vi "Echo_Handle_Frames_API.vi"(5 "frames":T1 {"flags" format="%.0x"; "id" format="%.0x"}, 7 "context":T2 {"ack hi" format="%.0x"; "ack lo" format="%.0x"; "test hi" format="%.0x"; "test lo" format="%.0x"}, 8 "error in (no error)":errorcluster, 9 "counters in":T3, 10 "time store in":T4, 11 "channel in":refnum<class "CANsub_Channel.lvclass">) -> (0 "error out":errorcluster, 1 "counters out":T3, 2 "time store out":T4, 3 "channel out":refnum<class "CANsub_Channel.lvclass">)   [LabVIEW 2021]
doc: "S5 echo via API: handles all frames of one Read: frames received += count; per frame Echo_Classify_API ? Test: Echo_Send_Echo_API, Ack: Echo_Send_Report, Other: nothing. Loop-safe: no allocation, bounded time."
uses:
  Echo_Time_Store.ctl
  Echo_Counters.ctl
  Echo_Context.ctl
  api/CANsub_Channel/CANsub_Channel.lvclass
  api/Typedefs/CANsub_Frames.ctl
  api/CANsub_API.lvlib
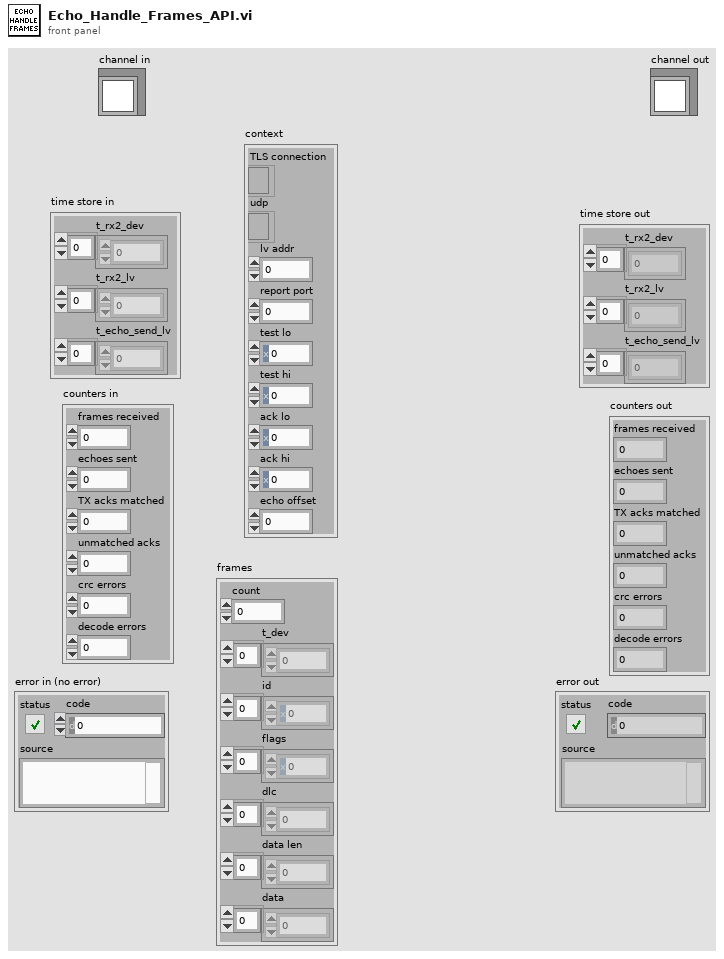
[diagram p1: front panel]
types:
  T1 = typedef "CANsub_API.lvlib/CANsub_Frames.ctl" = cluster{"count":i32, "t_dev":dbl[], "id":u32[], "flags":u16[], "dlc":u8[], "data len":u8[], "data":u8[]}
  T2 = typedef "Echo_Context.ctl" = cluster{"TLS connection":refnum<k5>, "udp":refnum<k16>, "lv addr":u32, "report port":u16, "test lo":u32, "test hi":u32, "ack lo":u32, "ack hi":u32, "echo offset":i32}
  T3 = typedef "Echo_Counters.ctl" = cluster{"frames received":u32, "echoes sent":u32, "TX acks matched":u32, "unmatched acks":u32, "crc errors":u32, "decode errors":i32}
  T4 = typedef "Echo_Time_Store.ctl" = cluster{"t_rx2_dev":dbl[], "t_rx2_lv":dbl[], "t_echo_send_lv":dbl[]}
  T5 = typedef "Echo_Frame.ctl" = cluster{"kind":T6, "id":u32, "t_dev":dbl, "seq":u16, "idx":u8, "key":i32, "index":i32}
  T6 = typedef "Echo_Frame_Kind.ctl" = enum16{"Other", "Test", "Ack"}
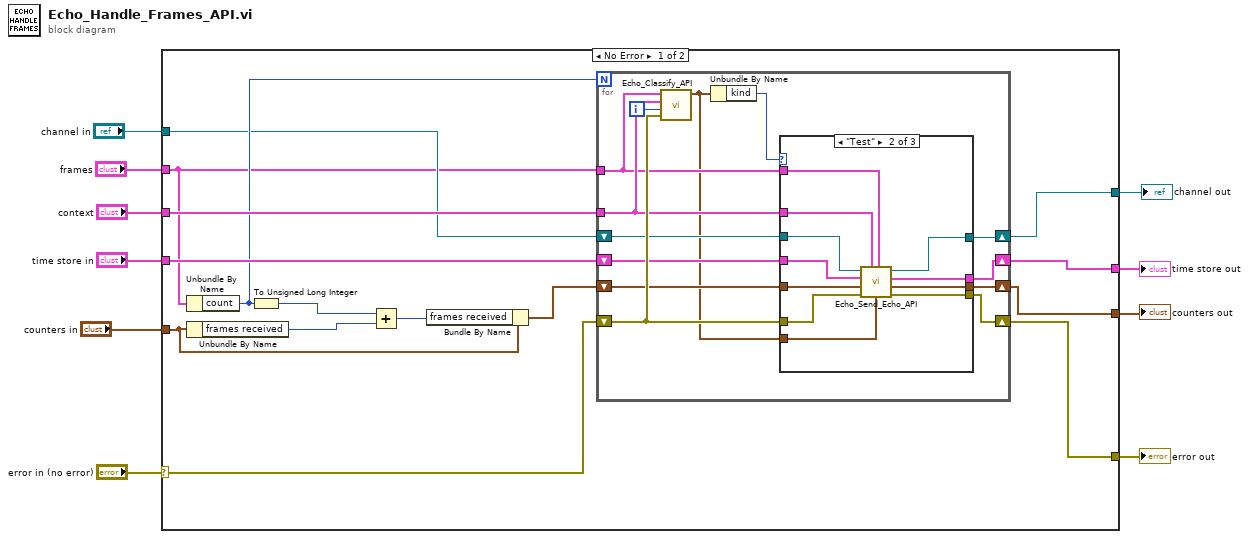
[diagram p0: block diagram]
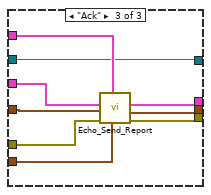
[diagram p3: hidden frame]
diagram:
  n1 = case shown="No Error" "error in (no error)" {
    selector: "error in (no error)" -> [w20 w66]
    tunnel: [w16 w66] -> w9
    tunnel: [w18 w65] -> w8
    tunnel: "time store in" -> [w22 w65]
    tunnel: [w17 w64] -> w6
    tunnel: "counters in" -> [w25 w64]
    tunnel: "context" -> [w19 _]
    tunnel: "frames" -> [w12 _]
    tunnel: "channel in" -> [w13 w63]
    tunnel: [w11 w63] -> w1
    frame No Error {
      n2 = Unbundle By Name(w12) -> ("count"=w14:i32)
      n3 = Unbundle By Name(w25) -> ("frames received"=w24:u32)
      n4 = To Unsigned Long Integer(number=w14) -> (unsigned 32bit integer=w15:u32)
      n5 = Add(x=w15, y=w24) -> (x+y=w23:u32)
      n6 = Bundle By Name(cluster=w25, "frames received"=w23) -> (w21:T3)
      n7 = for {
        N: w14 -> [_]
        shift-right: [w29] -> w11
        shift-left: w13 -> [w33]
        shift-right: [w28] -> w18
        shift-left: w22 -> [w32]
        shift-right: [w26] -> w17
        shift-left: w21 -> [w31]
        shift-right: [w27] -> w16
        shift-left: w20 -> [w36]
        tunnel: w12 -> [w34]
        tunnel: w19 -> [w35]
        i -> [w38]
        n8 = call "Echo_Classify_API.vi"("error in (no error)"=w36, "i"=w38, "context"=w35, "frames"=w34) -> ("frame"=w30:T5)  [unwired: 6 in, 1 out]
        n9 = Unbundle By Name(w30) -> ("kind"=w37:T6)
        n10 = case shown="\"Test\"" w37 {
          tunnel: [w42 w53 w54] -> w29
          tunnel: [w41 w52 w62] -> w28
          tunnel: [w40 w51 w61] -> w26
          tunnel: [w39 w50 w60] -> w27
          tunnel: w36 -> [w39 w49 w59]
          tunnel: w35 -> [_ w48 w57]
          tunnel: w34 -> [_ w47 _]
          tunnel: w33 -> [w42 w46 w54]
          tunnel: w32 -> [w41 w45 w56]
          tunnel: w31 -> [w40 w44 w58]
          tunnel: w30 -> [_ w43 w55]
          frame "Other", Default {
          }
          frame "Test" {
            n11 = call "Echo_Send_Echo_API.vi"("frames"=w47, "frame"=w43, "context"=w48, "error in (no error)"=w49, "counters in"=w44, "time store in"=w45, "channel in"=w46) -> ("error out"=w50:errorcluster, "counters out"=w51:T3, "time store out"=w52:T4, "channel out"=w53:refnum<class "CANsub_Channel.lvclass">)  [unwired: 1 in]
          }
          frame "Ack" {
            n12 = call "Echo_Send_Report.vi"("frame"=w55, "context"=w57, "error in (no error)"=w59, "counters in"=w58, "time store in"=w56) -> ("error out"=w60:errorcluster, "counters out"=w61:T3, "time store out"=w62:T4)  [unwired: 4 in]
          }
        }
      }
    }
    frame Error {
    }
  }
  "error out" <- w9
  "time store out" <- w8
  "counters out" <- w6
  "channel out" <- w1
